vi "Test_RX_Stats_Update.vi"(8 "error in (no error)":errorcluster, 9 "buffers in":T3, 10 "result":T1, 11 "stats in":T2 {"last data" format="%.0x"; "ids" format="%.0x"}) -> (0 "error out":errorcluster, 3 "stats out":T2 {"last data" format="%.0x"; "ids" format="%.0x"})   [LabVIEW 2021]
uses:
  C_RX_Buffers.ctl
  CANsub_C.lvlib
  typedefs/Test_RX_Stats.ctl
  C_Decode_Result.ctl
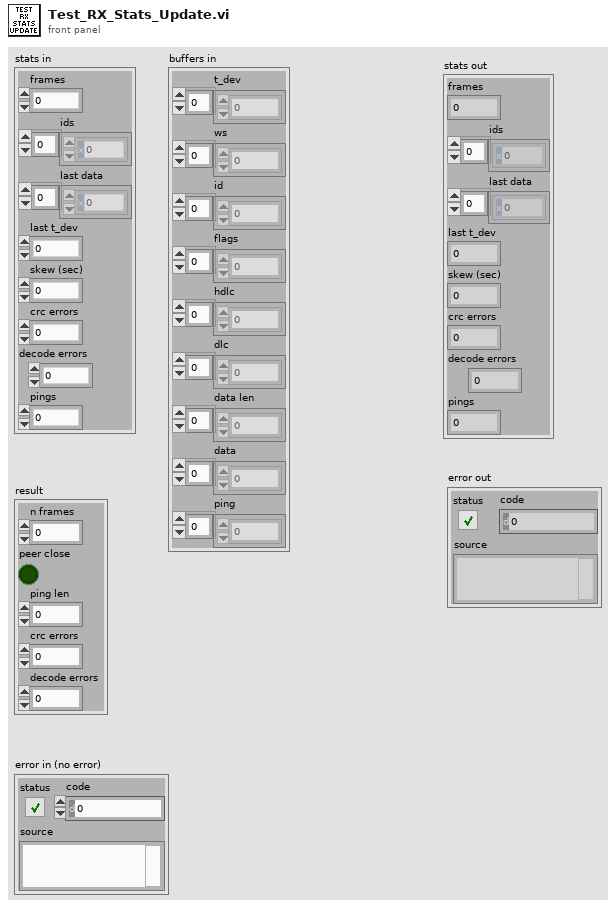
[diagram p1: front panel]
types:
  T1 = typedef "CANsub_C.lvlib/C_Decode_Result.ctl" = cluster{"n frames":i32, "peer close":bool, "ping len":i32, "crc errors":u32, "decode errors":i32}
  T2 = typedef "Test_RX_Stats.ctl" = cluster{"frames":i32, "ids":u32[], "last data":u8[], "last t_dev":dbl, "skew (sec)":dbl, "crc errors":u32, "decode errors":i32, "pings":i32}
  T3 = typedef "CANsub_C.lvlib/C_RX_Buffers.ctl" = cluster{"t_dev":dbl[], "ws":u8[], "id":u32[], "flags":u16[], "hdlc":u8[], "dlc":u8[], "data len":u8[], "data":u8[], "ping":u8[]}
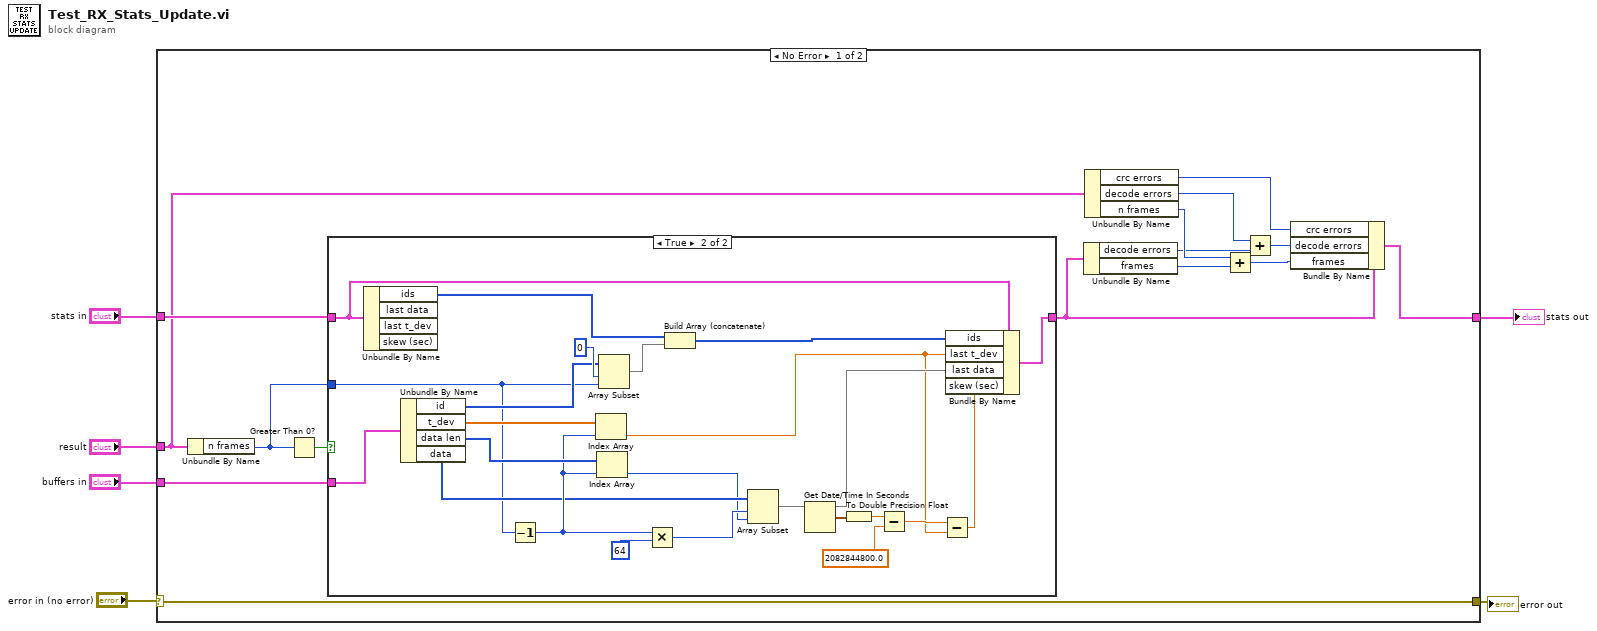
[diagram p0: block diagram]
diagram:
  n1 = case shown="No Error" "error in (no error)" {
    selector: "error in (no error)" -> [w17 w47]
    tunnel: "buffers in" -> [w21 _]
    tunnel: [w15 w46] -> w5
    tunnel: "stats in" -> [w20 w46]
    tunnel: "result" -> [w16 _]
    tunnel: [w17 w47] -> w1
    frame No Error {
      n2 = Unbundle By Name(w16) -> ("n frames"=w19:i32)
      n3 = Greater Than 0?(x=w19) -> (x > 0?=w18:bool)
      n4 = case shown="True" w18 {
        tunnel: w19 -> [_ w24]
        tunnel: w20 -> [w22 w23]
        tunnel: [w22 w42] -> w10
        tunnel: w21 -> [_ w41]
        frame False {
        }
        frame True {
          n5 = Unbundle By Name(w23) -> ("ids"=w39:u32[])  [unwired: 3 out]
          n6 = Unbundle By Name(w41) -> ("id"=w40:u32[], "t_dev"=w38:dbl[], "data len"=w37:u8[], "data"=w34:u8[])
          n7 = Decrement(x=w24) -> (x-1=w36:i32)
          n8 = Index Array(array=w38, index=w36) -> (element=w26:dbl)
          n9 = Index Array(array=w37, index=w36) -> (element=w32:u8)
          n10 = Array Subset(array=w40, index=0, length=w24) -> (w44:u32[])
          n11 = Multiply(x=w36, y=64 ("x")) -> (x*y=w33:i32)
          n12 = Build Array (concatenate)(w39, w44) -> (w43:u32[])
          n13 = Array Subset(array=w34, index=w33, length=w32) -> (w31:u8[])
          n14 = Get Date/Time In Seconds() -> (seconds since 1Jan1904=w30:timestamp)
          n15 = To Double Precision Float(number=w30) -> (double precision float=w29:dbl)
          n16 = Subtract(x=w29, y=2082844800.0) -> (x-y=w27:dbl)
          n17 = Subtract(x=w27, y=w26) -> (x-y=w25:dbl)
          n18 = Bundle By Name(cluster=w23, "ids"=w43, "last t_dev"=w26, "last data"=w31, "skew (sec)"=w25) -> (w42:T2)
        }
      }
      n19 = Unbundle By Name(w10) -> ("decode errors"=w12:i32, "frames"=w14:i32)
      n20 = Unbundle By Name(w16) -> ("crc errors"=w9:u32, "decode errors"=w11:i32, "n frames"=w13:i32)
      n21 = Add(x=w13, y=w14) -> (x+y=w7:i32)
      n22 = Add(x=w11, y=w12) -> (x+y=w8:i32)
      n23 = Bundle By Name(cluster=w10, "crc errors"=w9, "decode errors"=w8, "frames"=w7) -> (w15:T2)
    }
    frame Error {
    }
  }
  "stats out" <- w5
  "error out" <- w1
